vi "Highlight String Constant.vi"(8 "error in (no error)":errorcluster, 10 "Cluster":T1, 11 "JKI SM in":refnum<class "JKI SM.lvclass">) -> (0 "error out":errorcluster, 3 "JKI SM out":refnum<class "JKI SM.lvclass">)   [LabVIEW 2020]
uses:
  JKI State Machine API/source/JKI SM/JKI SM.lvclass
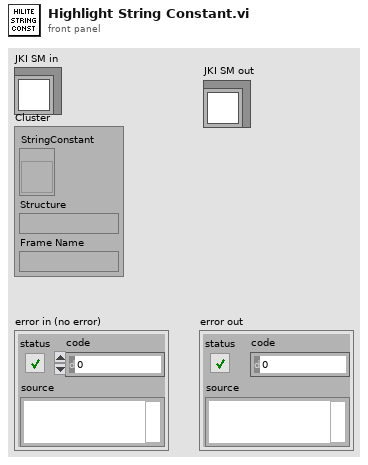
[diagram p1: front panel]
types:
  T1 = cluster{"StringConstant":refnum<vi>, "Structure":string, "Frame Name":string}
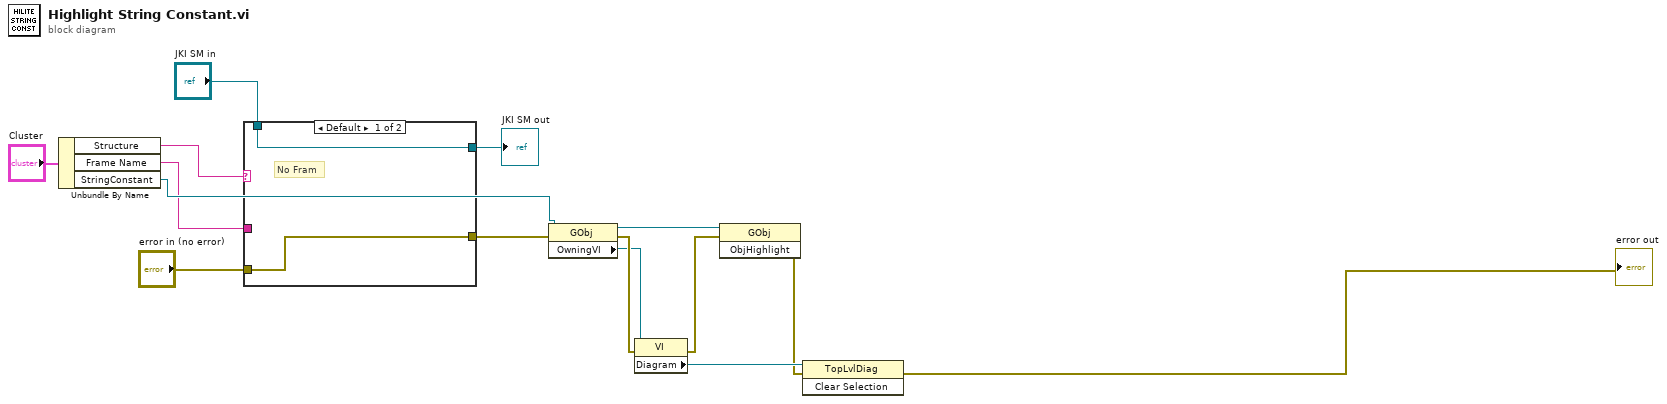
[diagram p0: block diagram]
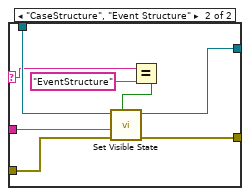
[diagram p2: hidden frame]
diagram:
  n1 = Unbundle By Name("Cluster") -> ("Structure"=w7:string, "Frame Name"=w8:string, "StringConstant"=w9:refnum<vi>)
  n2 = case shown="Default" w7 {
    selector: w7 -> [_ w19]
    tunnel: [w16 w25] -> w15
    tunnel: "error in (no error)" -> [w16 w24]
    tunnel: "JKI SM in" -> [w17 w23]
    tunnel: [w17 w22] -> w11
    tunnel: w8 -> [_ w21]
    frame Default {
      # "No Fram"
    }
    frame "CaseStructure", "Event Structure" {
      n3 = Equal?(x=w19, y="EventStructure") -> (x = y?=w18:bool)
      n4 = call "Set Visible State.vi"("Event Structure (F: Case Structure)"=w18, "error in (no error)"=w24, "State Name"=w21, "JKI SM in"=w23) -> ("error out"=w25:errorcluster, "JKI SM out"=w22:refnum<class "JKI SM.lvclass">)  [unwired: 6 in]
    }
  }
  "JKI SM out" <- w11
  n5 = property class="GObj"(reference=w9, error in=w15) -> (reference out=w1:refnum<vi>, error out=w4:errorcluster, "OwningVI"=w3:refnum<vi>)
  n6 = property class="VI"(reference=w3, error in=w4) -> (error out=w5:errorcluster, "Diagram"=w6:refnum<vi>)  [unwired: 1 out]
  n7 = invoke class="GObj" method="ObjHighlight"(reference=w1, error in=w5) -> (error out=w2:errorcluster)  [unwired: 1 in, 2 out]
  n8 = invoke class="TopLvlDiag" method="Clear Selection"(reference=w6, error in=w2) -> (error out=→"error out":errorcluster)  [unwired: 1 in, 2 out]
